vi "libssh2_exit.vi"(8 "error in (no error)":errorcluster) -> (0 "error out":errorcluster)   [LabVIEW 2017, in "libssh2.lvlib"]
doc: "Exit libssh2 and release internal resources."
uses:
  libssh2.lvlib
  Global Settings.vi
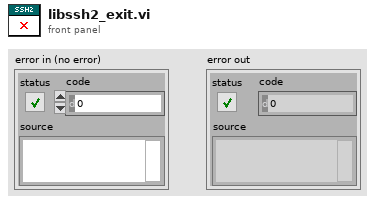
[diagram p1: front panel]
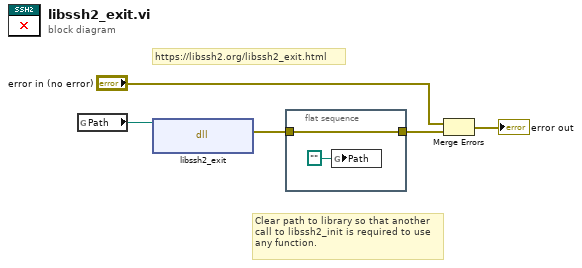
[diagram p0: block diagram]
diagram:
  # "Clear path to library so that another\ncall to libssh2_init is required to use\nany function."
  # "https://libssh2.org/libssh2_exit.html"
  n1 = global read "Global Settings.vi" "Path"() -> (w3:path)
  n2 = dll-call lib="?" fn="libssh2_exit"(path in=w3) -> (error out=w1:errorcluster)  [unwired: 3 in, 1 out]
  n3 = flat-sequence {
    tunnel: [w7] -> w2
    tunnel: w1 -> [w7]
    frame #0 {
      n4 = global write "Global Settings.vi" "Path"(path "") -> ()
    }
  }
  n5 = Merge Errors("error in (no error)", w2) -> (→"error out":errorcluster)
